vi "Servo.vi"(8 "error in (no error)":errorcluster, 9 "Angulo":u8 max=180 format="%x", 10 "Canal":u8 format="%x", 11 "VISA resource name":refnum<visa-resource-name>) -> (0 "error out":errorcluster, 2 "respuesta":string, 3 "VISA resource name out":refnum<visa-resource-name>)   [LabVIEW 2026]
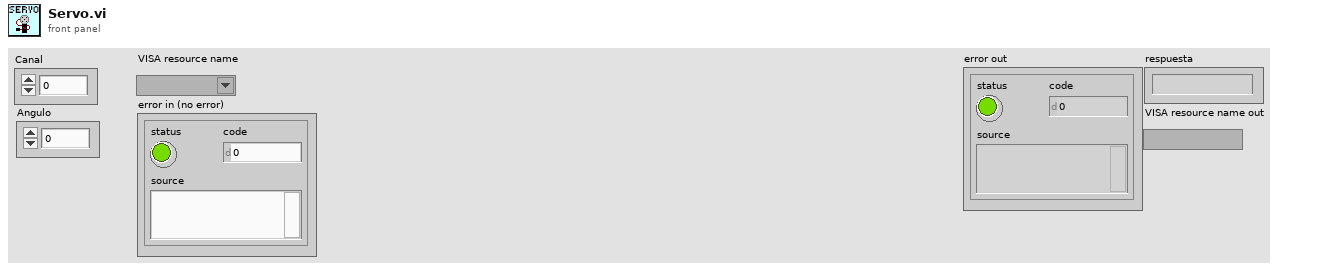
[diagram p1: front panel]
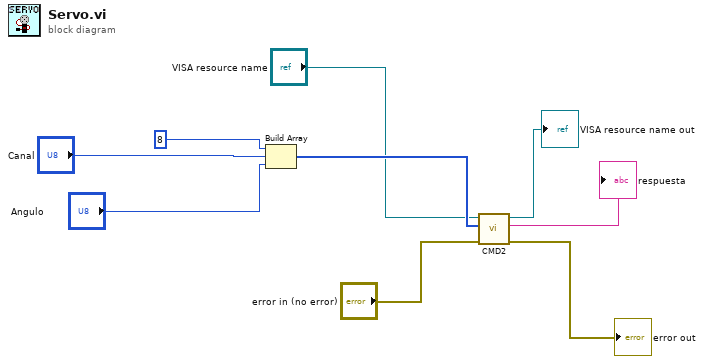
[diagram p0: block diagram]
diagram:
  n1 = Build Array(u8 8, "Canal", "Angulo") -> (w8:u8[])
  n2 = call "CMD2.vi"("error in (no error)"="error in (no error)", "Comando"=w8, "VISA resource name"="VISA resource name") -> ("error out"=→"error out":errorcluster, "respuesta"=→"respuesta":string, "VISA resource name out"=→"VISA resource name out":refnum<visa-resource-name>)  [unwired: 6 in]
